vi "Posicions inicials depredadors.vi"(11 "# dep":i32) -> (2 "y":dbl[](array[numeric]), 3 "x":dbl[](array[numeric]))   [LabVIEW 2023]
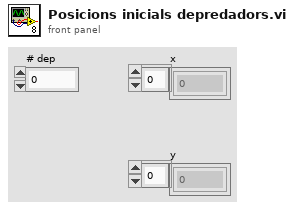
[diagram p1: front panel]
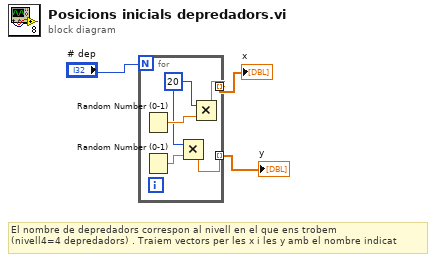
[diagram p0: block diagram]
diagram:
  # "El nombre de depredadors correspon al nivell en el que ens trobem\n(nivell4=4 depredadors) . Traiem vectors per les x i les y amb el nombre indicat"
  n1 = for {
    N: "# dep" -> [_]
    tunnel: [w5] -> w2 mode=indexing
    tunnel: [w4] -> w3 mode=indexing
    w6 = 20
    n2 = Random Number (0-1)() -> (number: 0 to 1=w8:dbl)
    n3 = Random Number (0-1)() -> (number: 0 to 1=w7:dbl)
    n4 = Multiply(x=w6, y=w7) -> (x*y=w4:dbl)
    n5 = Multiply(x=w6, y=w8) -> (x*y=w5:dbl)
  }
  "y" <- w3
  "x" <- w2
